vi "W32B Ensure Folder.vi"(0 "folder":path, 11 "error in":errorcluster) -> (4 "folder out":path, 15 "error out":errorcluster)   [LabVIEW 2020]
doc: "Creates folder when it does not exist yet (one level - its parent must exist) and passes the path on. Nothing happens when error in carries an error."
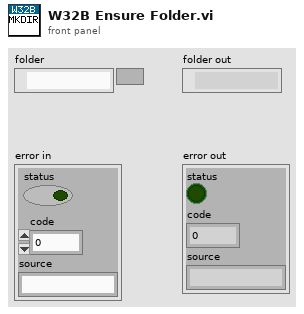
[diagram p1: front panel]
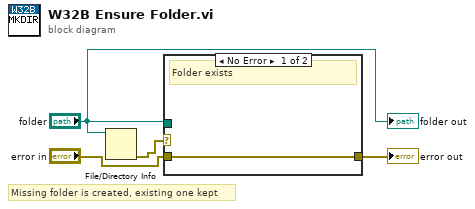
[diagram p0: block diagram]
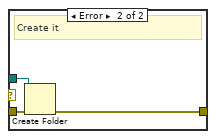
[diagram p2: hidden frame]
diagram:
  # "Missing folder is created, existing one kept"
  n1 = File/Directory Info(path="folder") -> (error out=w4:errorcluster)  [unwired: 1 in, 6 out]
  n2 = case shown="No Error" w4 {
    tunnel: "error in" -> [w5 w6]
    tunnel: "folder" -> [_ w7]
    tunnel: [w5 w8] -> w3
    frame No Error {
      # "Folder exists"
    }
    frame Error {
      # "Create it"
      n3 = Create Folder(path (use dialog)=w7, error in=w6) -> (error out=w8:errorcluster)  [unwired: 1 in, 2 out]
    }
  }
  "error out" <- w3
  "folder out" <- "folder"
